vi "RDC-permittivity-Advanced.vi"(7 "basic data(open, short, water)":T1[](array[typedef]), 11 "Common Format":T1) -> (3 "Common Format out":T1)   [LabVIEW 2020, in "RDC-Reflection_Data_Computation.lvlib"]
doc: "Computes the permittivity of a Common Format cluster with the Advance method from the basic data (open, short, water), using RDC-Array-calc_cf_c0_m1."
uses:
  RDC-Reflection_Data_Computation.lvlib
  Reflector/RFH-common_data_format.ctl
  Reflector/RFH-Reflection_File_Handler.lvlib
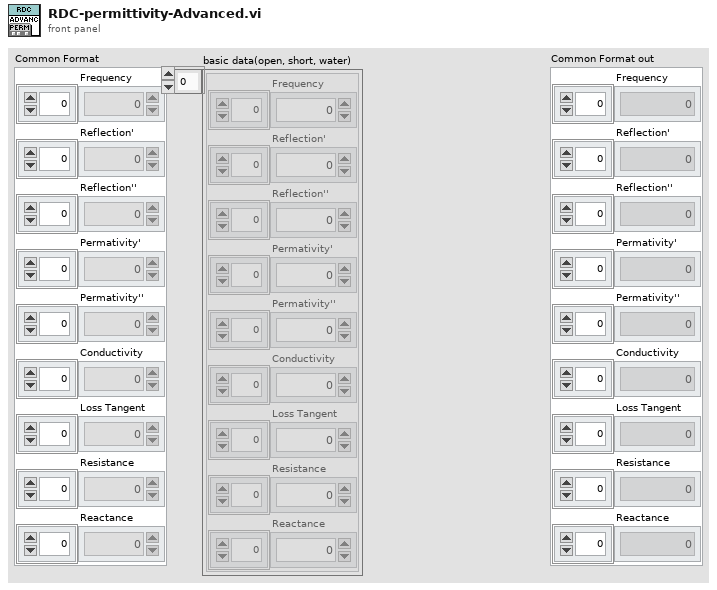
[diagram p1: front panel]
types:
  T1 = typedef "RFH-Reflection_File_Handler.lvlib/RFH-common_data_format.ctl" = cluster{"Frequency":dbl[], "Reflection'":dbl[], "Reflection''":dbl[], "Permativity'":dbl[], "Permativity''":dbl[], "Conductivity":dbl[], "Loss Tangent":dbl[], "Resistance":dbl[], "Reactance":dbl[]}
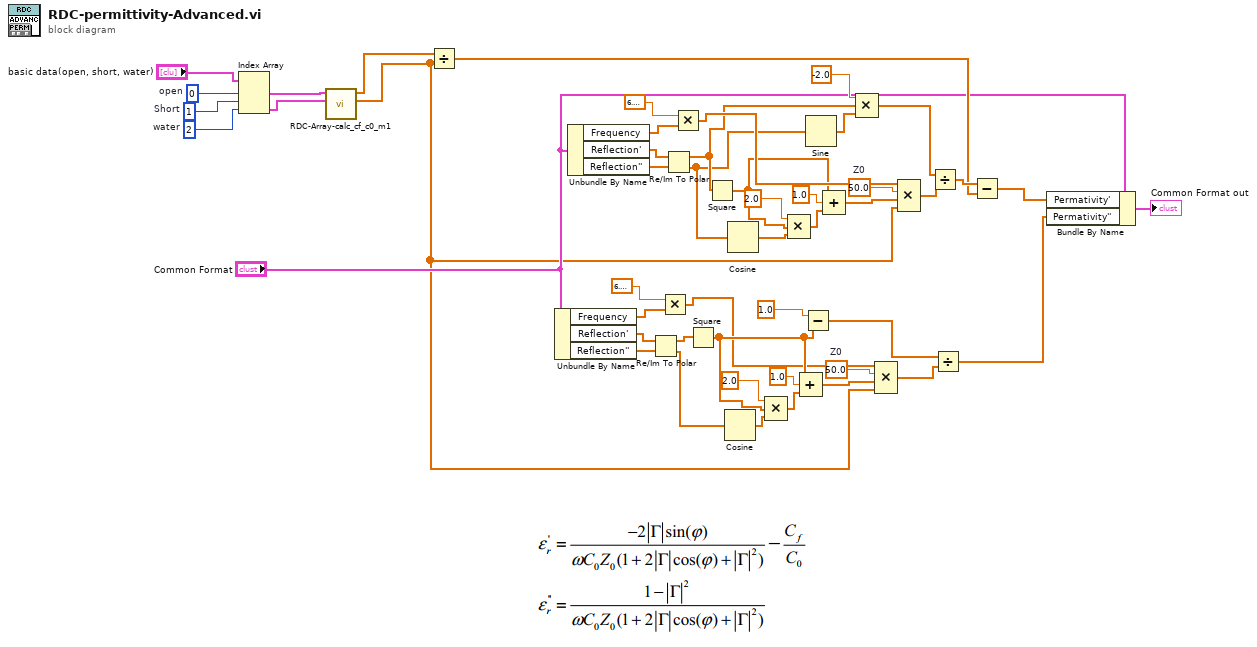
[diagram p0: block diagram]
diagram:
  w24 = 50.0  # Z0
  w33 = 50.0  # Z0
  w46 = 2  # water
  w47 = 1  # Short
  w48 = 0  # open
  n1 = Index Array(array="basic data(open, short, water)", index #1=w48, index #2=w47, index #3=w46) -> (element #1=w5:T1, element #3=w2:T1)  [unwired: 1 out]
  n2 = call "RDC-Array-calc_cf_c0_m1.vi"("water"=w2, "Open"=w5) -> ("C0"=w3:dbl[], "cf"=w4:dbl[])  [unwired: 8 in]
  n3 = Divide(x=w4, y=w3) -> (x/y=w9:dbl[])
  n4 = Unbundle By Name("Common Format") -> ("Frequency"=w29:dbl[], "Reflection'"=w45:dbl[], "Reflection''"=w44:dbl[])
  n5 = Unbundle By Name("Common Format") -> ("Frequency"=w28:dbl[], "Reflection'"=w16:dbl[], "Reflection''"=w17:dbl[])
  n6 = Re/Im To Polar(2:w44, 3:w45) -> (0:w39:dbl[], 1:w43:dbl[])
  n7 = Multiply(x=6.283185307179586, y=w29) -> (x*y=w30:dbl[])
  n8 = Re/Im To Polar(2:w17, 3:w16) -> (0:w13:dbl[], 1:w14:dbl[])
  n9 = Multiply(x=6.283185307179586, y=w28) -> (x*y=w27:dbl[])
  n10 = Square(x=w43) -> (x^2=w37:dbl[])
  n11 = Square(x=w14) -> (x^2=w20:dbl[])
  n12 = Cosine(x=w39) -> (cos(x)=w38:dbl[])
  n13 = Cosine(x=w13) -> (cos(x)=w19:dbl[])
  n14 = Compound Arithmetic op=MULTIPLY(2.0, w37, w38) -> (w35:dbl[])
  n15 = Compound Arithmetic op=MULTIPLY(2.0, w20, w19) -> (w22:dbl[])
  n16 = Compound Arithmetic op=ADD(w37, 1.0, w35) -> (w34:dbl[])
  n17 = Subtract(x=1.0, y=w37) -> (x-y=w41:dbl[])
  n18 = Sine(x=w13) -> (sin(x)=w12:dbl[])
  n19 = Compound Arithmetic op=ADD(w20, 1.0, w22) -> (w23:dbl[])
  n20 = Compound Arithmetic op=MULTIPLY(-2.0, w14, w12) -> (w11:dbl[])
  n21 = Compound Arithmetic op=MULTIPLY(w30, w33, w34, w3) -> (w31:dbl[])
  n22 = Compound Arithmetic op=MULTIPLY(w27, w24, w23, w3) -> (w26:dbl[])
  n23 = Divide(x=w11, y=w26) -> (x/y=w10:dbl[])
  n24 = Divide(x=w41, y=w31) -> (x/y=w1:dbl[])
  n25 = Subtract(x=w10, y=w9) -> (x-y=w8:dbl[])
  n26 = Bundle By Name(cluster="Common Format", "Permativity'"=w8, "Permativity''"=w1) -> (→"Common Format out":T1)
